vi "Hide_window.vi"(8 "error in (no error)":errorcluster, 11 "State":T1(ring)=enum."Hidden") -> (0 "error out":errorcluster)   [LabVIEW 2021]
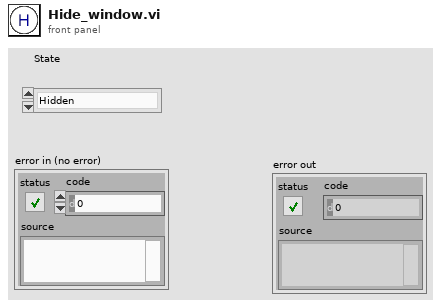
[diagram p1: front panel]
types:
  T1 = enum32{"Invalid", "Standard", "Closed", "Hidden", "Minimized", "Maximized"}
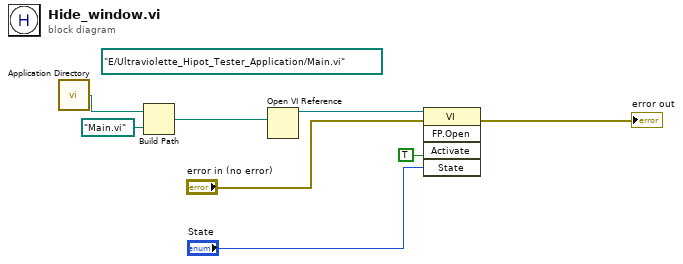
[diagram p0: block diagram]
diagram:
  (unwired) path "E:/Ultraviolette_Hipot_Tester_Application/Main.vi" ("vi path")
  n1 = call <vilib>:"Application Directory.vi"() -> ("Application Directory"=w3:path)
  n2 = Build Path(base path=w3, name or relative path=path "Main.vi") -> (appended path=w1:path)
  n3 = Open VI Reference(vi path=w1) -> (vi reference=w8:refnum<vi>)  [unwired: 5 in, 1 out]
  n4 = invoke class="VI" method="FP.Open"(reference=w8, error in="error in (no error)", "Activate"=TRUE ("Activate?"), "State"="State") -> (error out=→"error out":errorcluster)  [unwired: 1 in, 4 out]
